vi "DNL_Result.vi"(11 "Error In":errorcluster) -> (3 "Min DNL Code":i32, 4 "Max DNL Code":i32, 6 "Max DNL":dbl, 8 "DNL Plot":cluster{"X":i32, "Y":dbl}[](graph), 10 "Min DNL":dbl, 15 "Error Out":errorcluster)   [LabVIEW 2026, in "Core.lvlib"]
doc: "Displays and summarizes the results of a DNL measurement test, including graphical visualization and worst-case DNL statistics."
uses:
  Core.lvlib
  TypeDefs/Enum_Events.ctl
  TypeDefs/Enum_Event_Options.ctl
  TypeDefs/Enum_Notifier_Name.ctl
  TypeDefs/Enum_Notifier_Options.ctl
panel:
  out "Total":i32
  out "Values":i32 caption="Currently processing value index:"
  # "/"
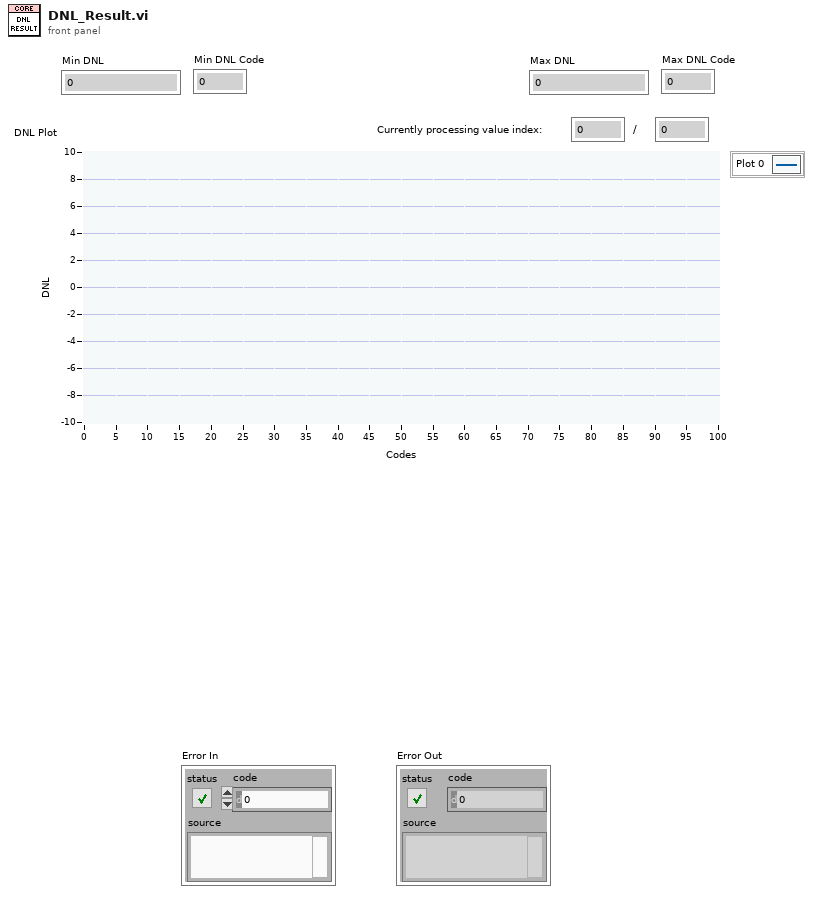
[diagram p1: front panel]
types:
  T1 = typedef "Core.lvlib/Enum_Notifier_Options.ctl" = enum16{"Create", "Send", "Status", "Release"}
  T2 = typedef "Core.lvlib/Enum_Notifier_Name.ctl" = enum16{"Device Type", "Test", "Instrument Spec", "Measurement Spec", "Status"}
  T3 = typedef "Core.lvlib/Enum_Event_Options.ctl" = enum16{"Create", "Generate", "Event Ref", "Destroy"}
  T4 = typedef "Core.lvlib/Enum_Events.ctl" = enum16{"Stop All", "Stop Subpanel", "Stop Test Spec", "Stop Result"}
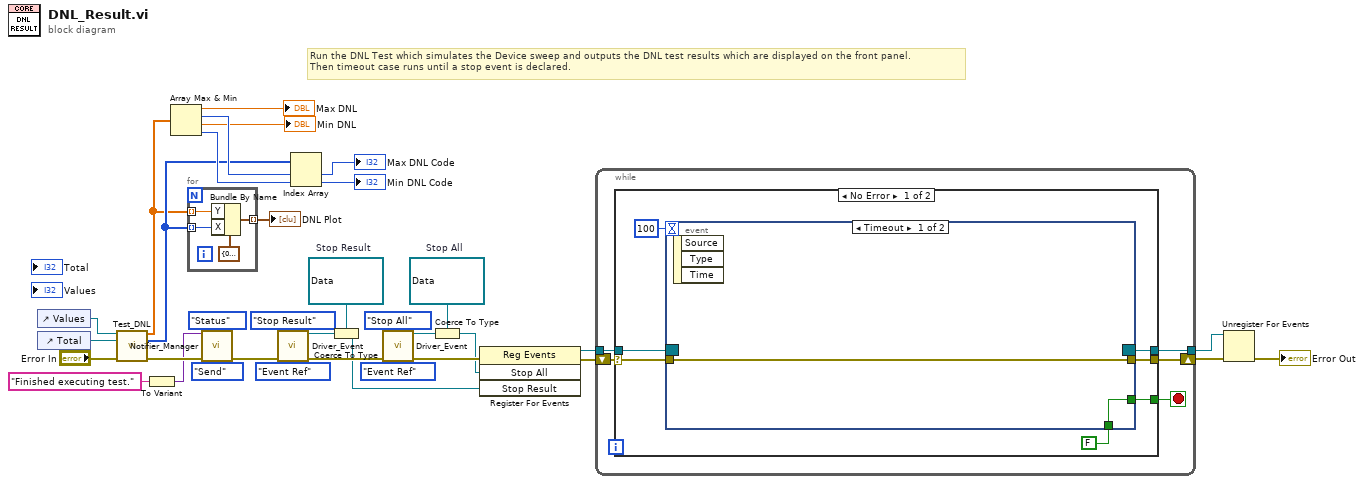
[diagram p0: block diagram]
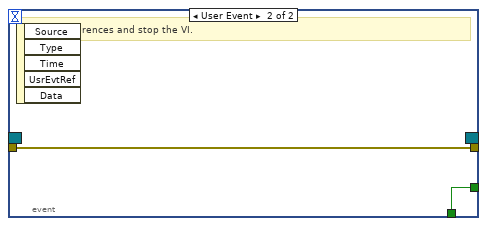
[diagram p2: hidden frame]
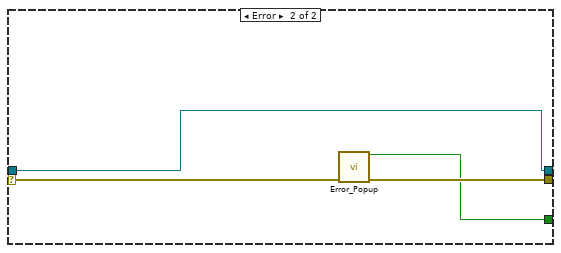
[diagram p3: hidden frame]
diagram:
  w17 = refnum<user-event> refnum  # Stop Result
  w19 = refnum<user-event> refnum  # Stop All
  # "Run the DNL Test which simulates the Device sweep and outputs the DNL test results which are displayed on the front panel.\nThen timeout case runs until a stop event is declared."
  n1 = control-ref of="Values"() -> (w2:refnum<vi>)
  n2 = control-ref of="Total"() -> (w1:refnum<vi>)
  n3 = call "Test_DNL.vi"("Values"=w2, "Total"=w1, "Error In"="Error In") -> ("DNL"=w4:dbl[], "Codes Array"=w5:i32[], "Error Out"=w11:errorcluster)  [unwired: 10 in]
  n4 = To Variant(anything="Finished executing test.") -> (Variant=w6:variant)
  n5 = Array Max & Min(array=w4) -> (max value=→"Max DNL":dbl, max index (indices)=w33:i32, min value=→"Min DNL":dbl, min index (indices)=w31:i32)
  n6 = for {
    tunnel: w4 -> [w38] mode=indexing
    tunnel: w5 -> [w37] mode=indexing
    tunnel: [w36] -> w3 mode=indexing
    n7 = Bundle By Name(cluster=cluster{"X":i32, "Y":dbl} {"X"=0, "Y"=0.0}, "Y"=w38, "X"=w37) -> (w36:cluster{"X":i32, "Y":dbl})
  }
  "DNL Plot" <- w3
  n8 = call "Notifier_Manager.vi"("Notifier Data"=w6, "Notifier Name"=Enum_Notifier_Name."Status", "Error In"=w11, "Notifier Options"=Enum_Notifier_Options."Send") -> ("Error Out"=w10:errorcluster)  [unwired: 10 in, 1 out]
  n9 = call "Driver_Event.vi"("Event"=Enum_Events."Stop Result", "Error In"=w10, "Event Operation"=Enum_Event_Options."Event Ref") -> ("Event Ref"=w21:refnum<user-event>, "Error Out"=w24:errorcluster)  [unwired: 11 in]
  n10 = Index Array(array=w5, index #1=w33, index #2=w31) -> (element #1=→"Max DNL Code":i32, element #2=→"Min DNL Code":i32)
  n11 = Coerce To Type(0:w21, 1:w17) -> (2:w18:refnum<user-event>)
  n12 = call "Driver_Event.vi"("Event"=Enum_Events."Stop All", "Error In"=w24, "Event Operation"=Enum_Event_Options."Event Ref") -> ("Event Ref"=w22:refnum<user-event>, "Error Out"=w23:errorcluster)  [unwired: 11 in]
  n13 = Coerce To Type(0:w22, 1:w19) -> (2:w20:refnum<user-event>)
  n14 = register-events(error in=w23, w20, w18) -> (reference out=w15:refnum<event-registration>, error out=w16:errorcluster)  [unwired: 1 in]
  n15 = while {
    tunnel: w15 -> [w41]
    shift-right: [w43] -> w14
    shift-left: w16 -> [w44]
    tunnel: [w40] -> w12
    stop <- w42 stop-if-true
    n16 = case shown="No Error" w44 {
      selector: w44 -> [w50 w59]
      tunnel: [w49 w58] -> w43
      tunnel: [w48 w57] -> w42
      tunnel: w41 -> [w46 w56]
      tunnel: [w45 w56] -> w40
      frame No Error {
        n17 = event shown="[0] Timeout" {
          selector: w46 -> [_ _]
          dyn-events: [_ _] -> w45
          timeout: 100 -> [_ _]
          tunnel: w50 -> [w53 w55]
          tunnel: [w53 w55] -> w49
          tunnel: [w52 w54] -> w48
          tunnel: FALSE -> [w52 w54]
          event Timeout {
            n18 = event-data() -> ()  [unwired: 1 in, 3 out]
          }
          event User Event {
            # "Close all references and stop the VI."
            n19 = event-data() -> ()  [unwired: 1 in, 5 out]
          }
        }
      }
      frame Error {
        n20 = call "Error_Popup.vi"("Error In"=w59) -> ("Stop?"=w57:bool, "Error Out"=w58:errorcluster)  [unwired: 13 in]
      }
    }
  }
  n21 = Unregister For Events(event registration refnum=w12, error in=w14) -> (error out=→"Error Out":errorcluster)
